vi "Do_Inspect_R.vi"(0 "VISA Refnum in":refnum<visa-resource-name>, 3 "connection ID":refnum<k5>, 4 "Recipe":T1, 5 "error in (no error)":errorcluster) -> (2 "Dark Pixels":i16, 6 "Pitch (mm)":dbl[](array[numeric]), 7 "Width (mm)":dbl, 8 "Pin Count":i32, 9 "Part ID":u32, 10 "TCP Network Connection out":refnum<k5>, 11 "Surface Defect":string, 12 "Pins OK":bool, 13 "Surface OK":bool, 14 "VISA Refnum out":refnum<visa-resource-name>, 15 "Defect":string, 16 "Width Defect":string, 17 "Width OK":bool, 18 "Part OK":bool, 19 "error out":errorcluster)   [LabVIEW 2018]
uses:
  08_Alarm/Recipe.ctl
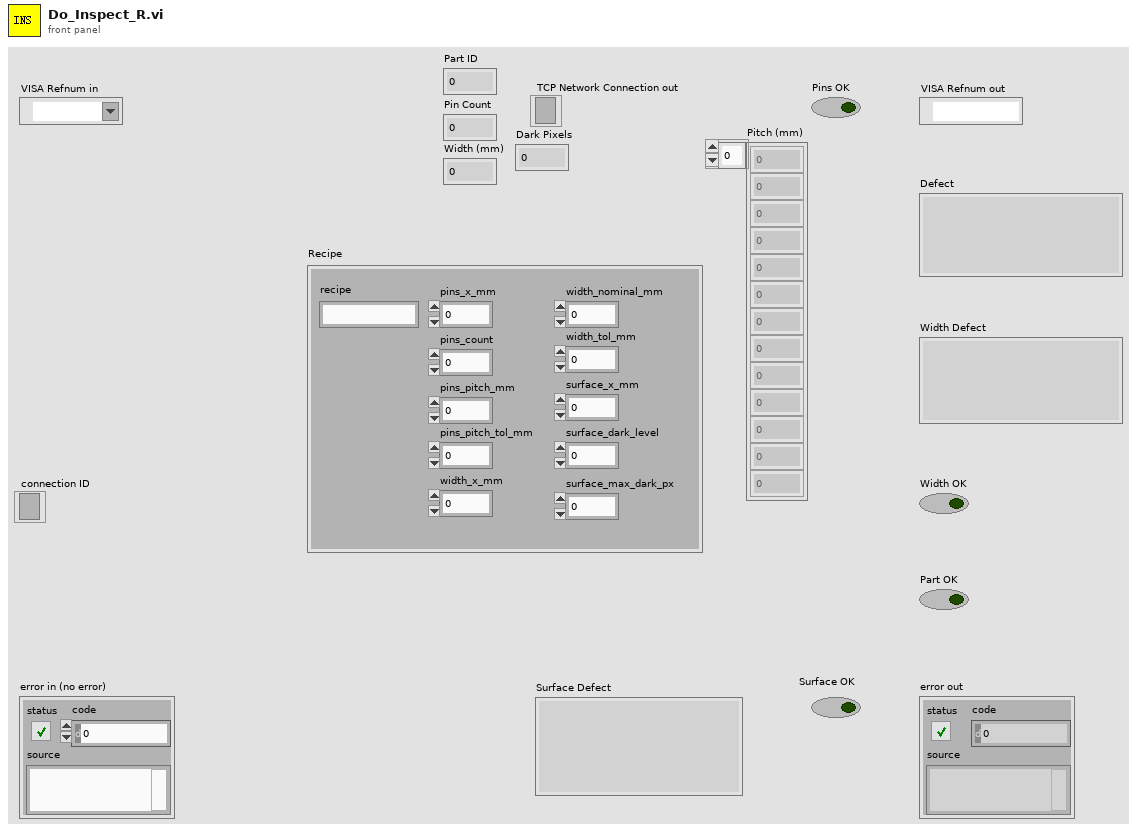
[diagram p1: front panel]
types:
  T1 = typedef "Recipe.ctl" = cluster{"recipe":string, "pins_x_mm":dbl, "pins_count":i32, "pins_pitch_mm":dbl, "width_x_mm":dbl, "width_nominal_mm":dbl, "surface_max_dark_px":i32, "surface_dark_level":dbl, "surface_x_mm":dbl, "width_tol_mm":dbl, "pins_pitch_tol_mm":dbl}
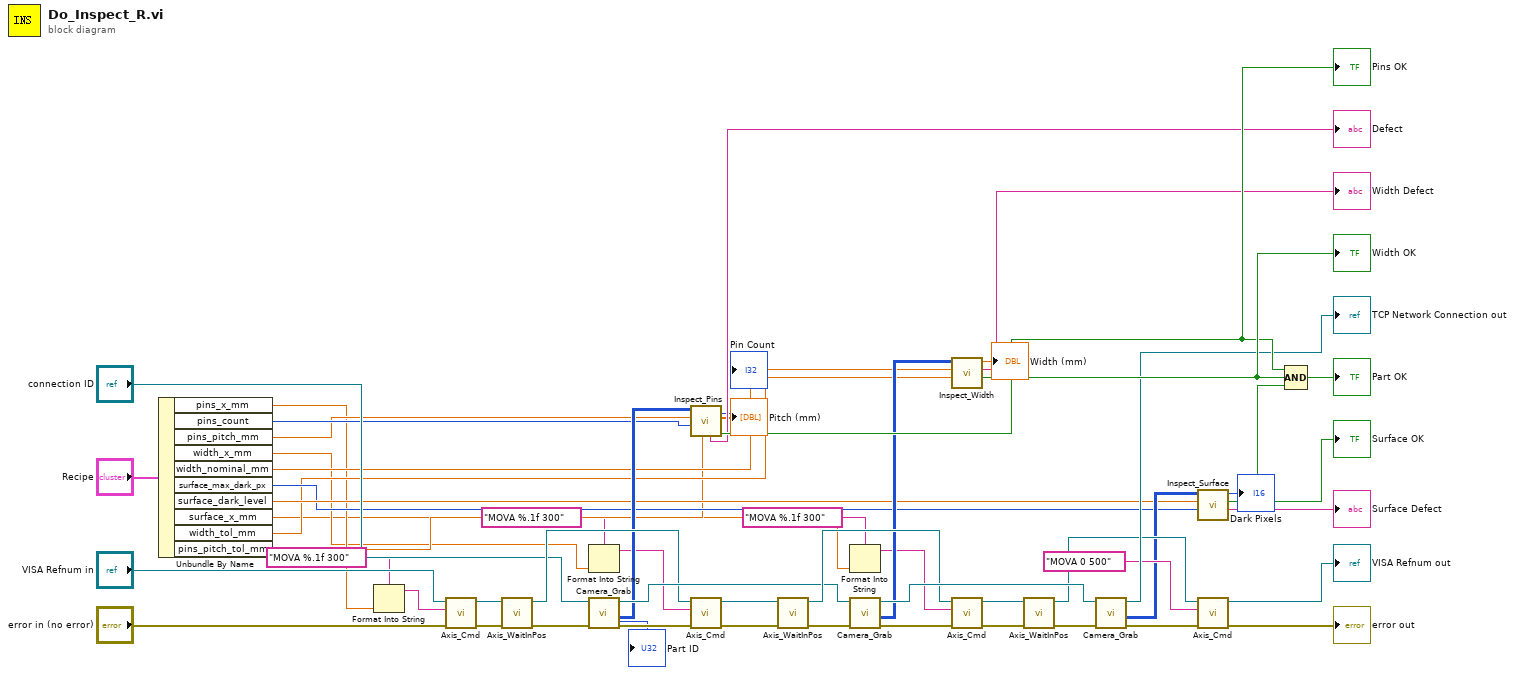
[diagram p0: block diagram]
diagram:
  n1 = Unbundle By Name("Recipe") -> ("pins_x_mm"=w14:dbl, "pins_count"=w21:i32, "pins_pitch_mm"=w15:dbl, "width_x_mm"=w12:dbl, "width_nominal_mm"=w20:dbl, "surface_max_dark_px"=w18:i32, "surface_dark_level"=w19:dbl, "surface_x_mm"=w10:dbl, "width_tol_mm"=w17:dbl, "pins_pitch_tol_mm"=w16:dbl)
  n2 = Format Into String(format string="MOVA %.1f 300", w14) -> (resulting string=w13:string)  [unwired: 2 in, 1 out]
  n3 = call "Axis_Cmd.vi"("error in (no error)"="error in (no error)", "Command"=w13, "VISA Refnum name"="VISA Refnum in") -> ("error out"=w24:errorcluster, "VISA Refnum name out"=w23:refnum<visa-resource-name>)  [unwired: 6 in, 1 out]
  n4 = call "Axis_WaitInPos.vi"("error in (no error)"=w24, "VISA Refnum name"=w23) -> ("error out"=w25:errorcluster, "visa out"=w47:refnum<visa-resource-name>)  [unwired: 8 in]
  n5 = Format Into String(format string="MOVA %.1f 300", w12) -> (resulting string=w11:string)  [unwired: 2 in, 1 out]
  n6 = call "Camera_Grab.vi"("error in (no error)"=w25, "TCP Network Connection in"="connection ID") -> ("error out"=w48:errorcluster, "Image"=w26:u8[][], "TCP Network Connection out"=w49:refnum<k5>, "Part ID"=→"Part ID":u32)  [unwired: 4 in, 2 out]
  n7 = call "Inspect_Pins.vi"("Pitch Tol (mm)"=w16, "Expected Pin Count"=w21, "Nominal Pitch (mm)"=w15, "Image"=w26) -> ("Pins OK"=w53:bool, "Pitch (mm)"=→"Pitch (mm)":dbl[], "Defect"=→"Defect":string, "Pin Count"=→"Pin Count":i32)  [unwired: 1 in, 3 out]
  "Pins OK" <- w53
  n8 = call "Axis_Cmd.vi"("error in (no error)"=w48, "Command"=w11, "VISA Refnum name"=w47) -> ("error out"=w30:errorcluster, "VISA Refnum name out"=w29:refnum<visa-resource-name>)  [unwired: 6 in, 1 out]
  n9 = call "Axis_WaitInPos.vi"("error in (no error)"=w30, "VISA Refnum name"=w29) -> ("error out"=w33:errorcluster, "visa out"=w50:refnum<visa-resource-name>)  [unwired: 8 in]
  n10 = Format Into String(format string="MOVA %.1f 300", w10) -> (resulting string=w9:string)  [unwired: 2 in, 1 out]
  n11 = call "Camera_Grab.vi"("error in (no error)"=w33, "TCP Network Connection in"=w49) -> ("error out"=w51:errorcluster, "Image"=w37:u8[][], "TCP Network Connection out"=w52:refnum<k5>)  [unwired: 4 in, 3 out]
  n12 = call "Inspect_Width.vi"("Width Tol (mm)"=w17, "Nominal Width (mm)"=w20, "Image"=w37) -> ("Width OK"=w54:bool, "Width Defect"=→"Width Defect":string, "Width (mm)"=→"Width (mm)":dbl)  [unwired: 6 in]
  "Width OK" <- w54
  n13 = call "Axis_Cmd.vi"("error in (no error)"=w51, "Command"=w9, "VISA Refnum name"=w50) -> ("error out"=w32:errorcluster, "VISA Refnum name out"=w31:refnum<visa-resource-name>)  [unwired: 6 in, 1 out]
  n14 = call "Axis_WaitInPos.vi"("error in (no error)"=w32, "VISA Refnum name"=w31) -> ("error out"=w34:errorcluster, "visa out"=w42:refnum<visa-resource-name>)  [unwired: 8 in]
  n15 = call "Camera_Grab.vi"("error in (no error)"=w34, "TCP Network Connection in"=w52) -> ("error out"=w43:errorcluster, "Image"=w38:u8[][], "TCP Network Connection out"=→"TCP Network Connection out":refnum<k5>)  [unwired: 4 in, 3 out]
  n16 = call "Inspect_Surface.vi"("Max Dark Pixels"=w18, "Dark Level"=w19, "Image"=w38) -> ("Surface Defect"=→"Surface Defect":string, "Surface OK"=w55:bool, "Dark Pixels"=→"Dark Pixels":i16)  [unwired: 6 in]
  "Surface OK" <- w55
  n17 = call "Axis_Cmd.vi"("error in (no error)"=w43, "Command"="MOVA 0 500", "VISA Refnum name"=w42) -> ("error out"=→"error out":errorcluster, "VISA Refnum name out"=→"VISA Refnum out":refnum<visa-resource-name>)  [unwired: 6 in, 1 out]
  n18 = Compound Arithmetic op=AND(w53, w54, w55) -> (→"Part OK":bool)
